vi "set Marker Control Mode.vi"(8 "error in (no error)":errorcluster, 9 "Marker Index":i32, 10 "Marker Mode":T1, 11 "Keysight 9020A in":refnum<class "Keysight 9020A.lvclass">) -> (0 "error out":errorcluster, 3 "Keysight 9020A out":refnum<class "Keysight 9020A.lvclass">)   [LabVIEW 2023, in "Spectrum Analyzer.lvlib" / "Keysight 9020A.lvclass"]
uses:
  Keysight 9020A.lvclass
  Keysight 9020A.lvclass/Keysight 9020A.ctl
  TYPE DEFINITION/TYPE Marker Control Mode.ctl
  Spectrum Analyzer.lvlib
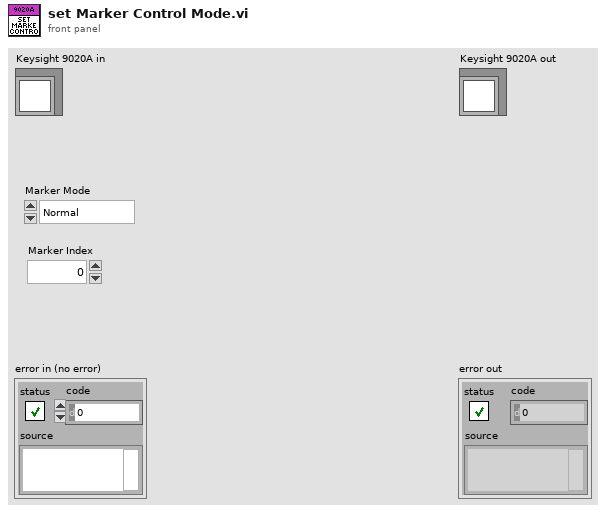
[diagram p1: front panel]
types:
  T1 = typedef "Spectrum Analyzer.lvlib/TYPE Marker Control Mode.ctl" = enum16{"Normal", "Delta", "Off"}
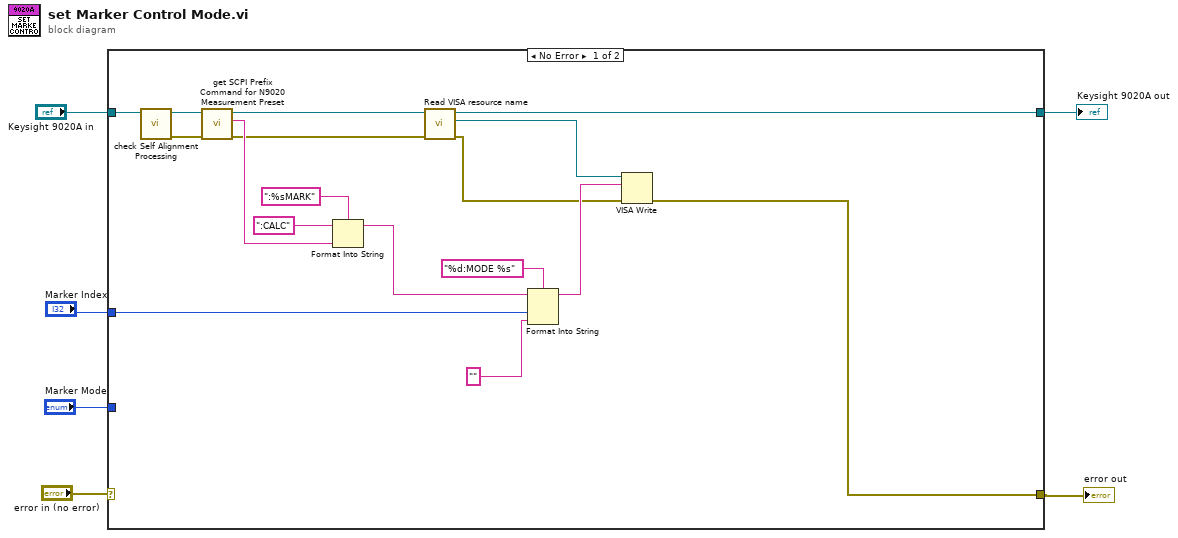
[diagram p0: block diagram]
diagram:
  n1 = case shown="No Error" "error in (no error)" {
    selector: "error in (no error)" -> [_ w24]
    tunnel: "Keysight 9020A in" -> [w13 w25]
    tunnel: [w14 w25] -> w5
    tunnel: [w21 w24] -> w1
    tunnel: "Marker Index" -> [w8 _]
    tunnel: "Marker Mode" -> [_ _]
    frame No Error {
      n2 = call "check Self Alignment Processing.vi"("Keysight 9020A in"=w13) -> ("error out"=w11:errorcluster, "Keysight 9020A out"=w12:refnum<class "Keysight 9020A.lvclass">)  [unwired: 8 in, 1 out]
      n3 = call "get SCPI Prefix Command for N9020 Measurement Preset.vi"("error in (no error)"=w11, "Keysight 9020A in"=w12) -> ("error out"=w10:errorcluster, "SCPI Prefix Command"=w17:string, "Keysight 9020A out"=w16:refnum<class "Keysight 9020A.lvclass">)  [unwired: 7 in]
      n4 = Format Into String(format string=":%sMARK", initial string=":CALC", w17) -> (resulting string=w15:string)  [unwired: 1 in, 1 out]
      n5 = call "Read VISA resource name.vi"("error in (no error)"=w10, "Keysight 9020A in"=w16) -> ("error out"=w9:errorcluster, "VISA resource name"=w20:refnum<visa-resource-name>, "Keysight 9020A out"=w14:refnum<class "Keysight 9020A.lvclass">)  [unwired: 7 in]
      n6 = Format Into String(format string="%d:MODE %s", initial string=w15, w8, "" ("input 2")) -> (resulting string=w23:string)  [unwired: 1 in, 1 out]
      n7 = VISA Write(VISA resource name=w20, write buffer=w23, error in (no error)=w9) -> (error out=w21:errorcluster)  [unwired: 2 out]
    }
    frame Error {
    }
  }
  "error out" <- w1
  "Keysight 9020A out" <- w5
